vi "VIH Utility - FILE - Remove Duplicated Paths from 1D Array.vi"(8 "error in":errorcluster, 11 "Array in":path[](array[path])) -> (0 "error out":errorcluster, 3 "Array out":path[](array[path]))   [LabVIEW 2014]
doc: "::: VI Helpeks :::\nCopyright (c) 2000-2026 Konstantin Shifershteyn. All rights reserved."
panel:
  # "VI Helpeks\nCopyright (c) 2012-2026 Konstantin Shifershteyn"
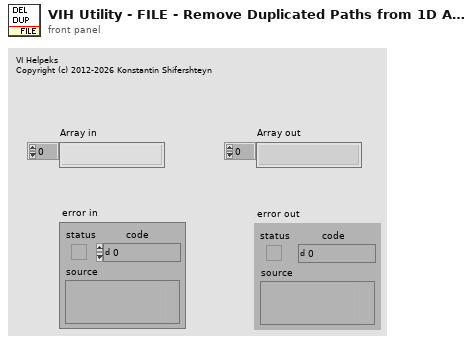
[diagram p1: front panel]
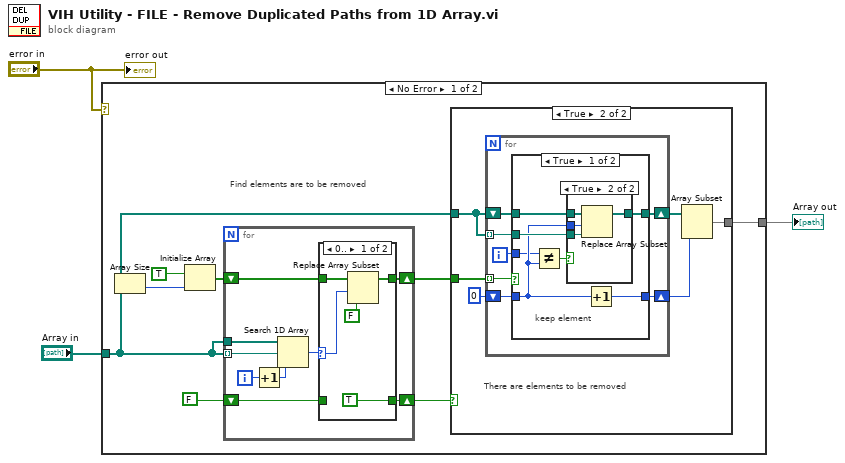
[diagram p0: block diagram]
diagram:
  n1 = case shown="No Error" "error in" {
    tunnel: [w10 w56] -> w1
    tunnel: "Array in" -> [w4 w56]
    frame No Error {
      # "Find elements are to be removed"
      n2 = Array Size(array=w4) -> (size(s)=w9:i32)
      n3 = Initialize Array(TRUE, w9) -> (w7:bool[])
      n4 = for {
        shift-right: [w43] -> w11
        shift-left: w7 -> [w44]
        tunnel: w4 -> [w48] mode=indexing
        tunnel: w4 -> [w47]
        shift-right: [w40] -> w5
        shift-left: FALSE -> [w41]
        i -> [w42]
        n5 = Increment(x=w42) -> (x+1=w46:i32)
        n6 = Search 1D Array(1D array=w47, element=w48, start index (0)=w46) -> (index of element=w45:i32)
        n7 = case shown="0.." w45 {
          selector: w45 -> [w52 _]
          tunnel: w44 -> [w53 w55]
          tunnel: [w51 w55] -> w43
          tunnel: w41 -> [_ w54]
          tunnel: [TRUE w54] -> w40
          frame 0.. {
            n8 = Replace Array Subset(array=w53, new element=FALSE, index=w52) -> (w51:bool[])
          }
          frame ..-1 {
          }
        }
      }
      n9 = case shown="True" w5 {
        tunnel: w11 -> [_ w15]
        tunnel: w4 -> [w12 w14]
        tunnel: [w12 w13] -> w10
        frame False {
        }
        frame True {
          # "There are elements to be removed"
          n10 = for {
            shift-right: [w23] -> w17
            shift-left: w14 -> [w24]
            tunnel: w15 -> [w25] mode=indexing
            shift-right: [w21] -> w16
            shift-left: 0 -> [w22]
            tunnel: w14 -> [w20] mode=indexing
            i -> [w19]
            n11 = case shown="True" w25 {
              tunnel: w24 -> [w31 w39]
              tunnel: [w30 w39] -> w23
              tunnel: w22 -> [w28 w38]
              tunnel: [w32 w38] -> w21
              tunnel: w20 -> [w29 _]
              tunnel: w19 -> [w27 _]
              frame True {
                # "keep element"
                n12 = Not Equal?(x=w27, y=w28) -> (x != y?=w26:bool)
                n13 = case shown="True" w26 {
                  tunnel: w31 -> [w33 w37]
                  tunnel: [w33 w36] -> w30
                  tunnel: w28 -> [_ w35]
                  tunnel: w29 -> [_ w34]
                  frame False {
                    # "no need\nto\noverwrite"
                  }
                  frame True {
                    n14 = Replace Array Subset(array=w37, new element=w34, index=w35) -> (w36:path[])
                  }
                }
                n15 = Increment(x=w28) -> (x+1=w32:i32)
              }
              frame False {
                # "element is to be removed"
              }
            }
          }
          n16 = Array Subset(array=w17, length=w16) -> (w13:path[])  [unwired: 1 in]
        }
      }
    }
    frame Error {
    }
  }
  "Array out" <- w1
  "error out" <- "error in"
